vi "Create Execution Unit.vi"(8 "error in":errorcluster, 10 "Item Ref":T2=18446744073709551615 format="%.0x", 11 "Execution Unit Factory Implementation in":refnum<class "Execution Unit Factory.lvclass">) -> (0 "error out":errorcluster, 1 "Asynchronous Execution Units":cluster{"Grouped Execution Units":T1[]}[](array[cluster]) {"Grouped Execution Units"."ReadWrite Channels" format="%.0x"; "Grouped Execution Units"."Outgoing Channels" format="%.0x"; "Grouped Execution Units"."Incoming Channels" format="%.0x"}, 2 "Inline Execution Units":T1[](array[typedef]) {"ReadWrite Channels" format="%.0x"; "Outgoing Channels" format="%.0x"; "Incoming Channels" format="%.0x"}, 3 "Execution Unit Factory Implementation out":refnum<class "Execution Unit Factory.lvclass">)   [LabVIEW 2020, in "Ballard ARINC 429 Engine.lvlib" / "Implementation.lvlib" / "Execution Unit Factory.lvclass"]
uses:
  Execution Unit Factory.lvclass
  Interfaces/Execution Unit/Execution Unit.lvclass
  <vilib>/NI VeriStand/Custom Device API/Custom Device Item Ref.ctl
  <vilib>/NI VeriStand/Custom Device API/Custom Device API.lvlib
  Interfaces/Controls/Execution Unit Information.ctl
  Interfaces/Interfaces.lvlib
  Rx Execution Unit/Rx Execution Unit.lvclass
  System Explorer/Implementation/Implementation.lvlib
  Tx Acyclic Labels Execution Unit/Tx Acyclic Labels Execution Unit.lvclass
  Scripting/Ballard/Ballard ARINC 429 Scripting.lvlib
  Custom Device/Custom Device.lvlib
  Tx Scheduled Labels Execution Unit/Tx Scheduled Labels Execution Unit.lvclass
  C:/Users/nitest/Desktop/Git 2020/niveristand-ballard-arinc429-custom-device/Source/Custom Device Support/Engine/Implementation/Execution Unit/Execution Unit.lvclass
  C:/Users/nitest/Desktop/Git 2020/niveristand-ballard-arinc429-custom-device/Source/Custom Device Support/Engine/Interfaces/Execution Unit/Execution Unit.lvclass
  C:/Users/nitest/Desktop/Git 2020/niveristand-ballard-arinc429-custom-device/Source/Custom Device Support/Engine/Implementation/Rx Execution Unit/Rx Execution Unit.lvclass
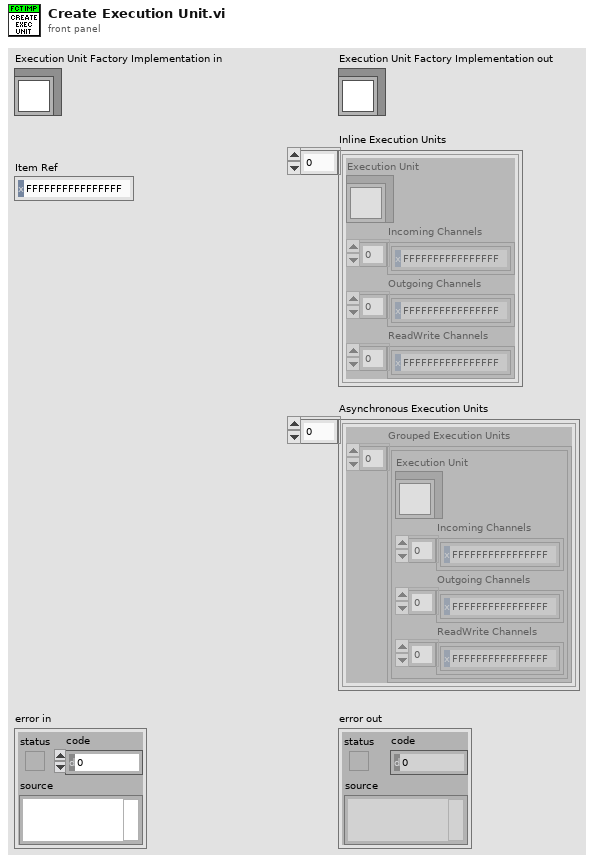
[diagram p1: front panel]
types:
  T1 = typedef "Ballard ARINC 429 Engine.lvlib/Interfaces.lvlib/Execution Unit Information.ctl" = cluster{"Execution Unit":refnum<class "Execution Unit.lvclass">, "Incoming Channels":T2[], "Outgoing Channels":T2[], "ReadWrite Channels":T2[]}
  T2 = typedef "Custom Device API.lvlib/Custom Device Item Ref.ctl" = u64
  T3 = typedef "RT Hardware Channel Settings.ctl" = cluster{"channel #":u16, "channel handle":u64, "labels settings for RT":T4[]}
  T4 = typedef "RT Label Settings.ctl" = cluster{"Name":string, "xmlName":string, "label":T5, "transfer period":u32, "SDI_Enabled":bool, "SDI":u8, "parameter driver data":T6, "transfer type":T9, "has timestamp?":bool, "Label Disable/Trigger Channel Reference":T2, "Message Handle":u64, "Initialized?":bool, "Word Initial Raw Value":u32, "Label Timestamp Channel Data Reference":T10, "disabled":bool}
  T5 = typedef "Label.ctl" = u8
  T6 = typedef "RT Parameters.ctl" = cluster{"parameter definitions":T7[], "Tx parameter refs":T2[]}
  T7 = typedef "Parameter Definition.ctl" = cluster{"start index":i32, "size":i32, "encoding":T8, "signed":bool, "scale multiplier":dbl, "scale offset":dbl}
  T8 = typedef "Encoding and Decoding.lvlib/Encoding.ctl" = enum16{"BNR", "BCD", "Discrete"}
  T9 = typedef "Transfer Type.ctl" = enum16{"Scheduled", "Acyclic", "Block", "Strobe"}
  T10 = typedef "Custom Device API.lvlib/Data Reference.ctl" = i32
  T11 = typedef "Rx Channel Data Offsets.ctl" = cluster{"error counts":u32, "rx execution time":i64}
  T12 = typedef "Custom Device API.lvlib/Custom Device Item Info.ctl" = cluster{"Name":string, "Is Channel":bool, "GUID":string, "Is Waveform":bool}
  T13 = cluster{"transfer type":T9, "Name":string, "hardware channel data":T3[], "Outgoing Channels":T2[], "ReadWrite Channels":T2[]}[]
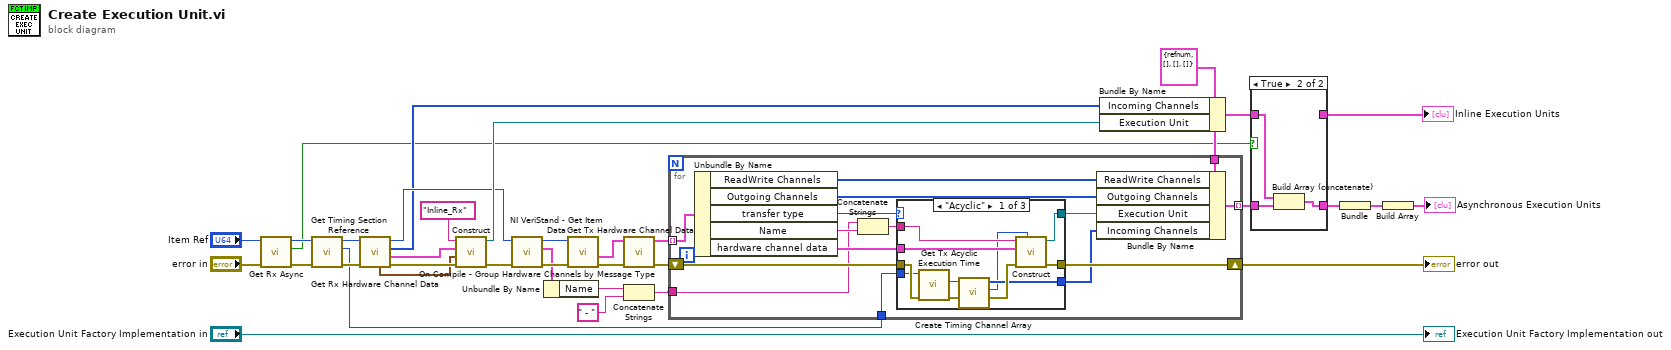
[diagram p0: block diagram]
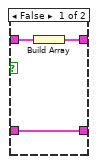
[diagram p2: hidden frame]
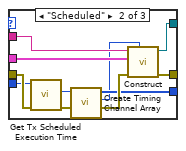
[diagram p3: hidden frame]
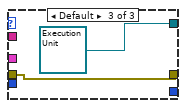
[diagram p4: hidden frame]
diagram:
  w23 = T1 {"Execution Unit"=refnum, "Incoming Channels"=[], "Outgoing Channels"=[], "ReadWrite Channels"=[]} ("Execution Unit Information")
  n1 = call "Get Rx Async.vi"("error in"="error in", "Ballard ARINC 429 custom device in"="Item Ref") -> ("error out"=w7:errorcluster, "rx async?"=w5:bool, "Ballard ARINC 429 custom device out"=w8:T2)  [unwired: 7 in]
  n2 = call "Get Timing Section Reference.vi"("error in"=w7, "Ballard ARINC 429 ref"=w8) -> ("error out"=w12:errorcluster, "timing section ref"=w9:T2, "Ballard ARINC 429 ref out"=w11:T2)  [unwired: 6 in, 1 out]
  n3 = call "Get Rx Hardware Channel Data.vi"("error in"=w12, "custom device ref in"=w11) -> ("error out"=w28:errorcluster, "Rx hardware channel data"=w29:T3[], "incoming channels"=w14:T2[], "custom device ref out"=w21:T2, "channel data offsets"=w13:T11)  [unwired: 5 in]
  n4 = call "Construct.vi"("error in"=w28, "channel data offsets"=w13, "RT hardware channels"=w29, "ID"="Inline_Rx") -> ("error out"=w22:errorcluster, "Ballard ARINC-429 Rx Execution Unit"=w27:refnum<class "Rx Execution Unit.lvclass">)  [unwired: 6 in]
  n5 = call <vilib>:"NI VeriStand - Get Item Data.vi"("error in (no error)"=w22, "Item Ref in"=w21) -> ("error out"=w19:errorcluster, "Item Info"=w18:T12, "Item Ref out"=w20:T2)  [unwired: 6 in, 1 out]
  n6 = Unbundle By Name(w18) -> ("Name"=w17:string)
  n7 = call "Get Tx Hardware Channel Data.vi"("error in"=w19, "custom device ref in"=w20) -> ("error out"=w31:errorcluster, "Tx hardware channel data"=w30:T3[])  [unwired: 6 in, 2 out]
  n8 = call "On Compile - Group Hardware Channels by Message Type.vi"("error in"=w31, "hardware channel data"=w30) -> ("error out"=w26:errorcluster, "hardware channel data by transfer type"=w24:T13)  [unwired: 8 in]
  n9 = Concatenate Strings(w17, " - " ("string")) -> (w15:string)
  n10 = for {
    shift-right: [w49] -> w25
    shift-left: w26 -> [w50]
    tunnel: w24 -> [w48] mode=indexing
    tunnel: w23 -> [w46]
    tunnel: [w44] -> w2 mode=indexing
    tunnel: w15 -> [w39]
    tunnel: w9 -> [w37]
    n11 = Unbundle By Name(w48) -> ("ReadWrite Channels"=w43:T2[], "Outgoing Channels"=w42:T2[], "transfer type"=w45:T9, "Name"=w40:string, "hardware channel data"=w41:T3[])
    n12 = Concatenate Strings(w39, w40) -> (w38:string)
    n13 = case shown="\"Acyclic\"" w45 {
      tunnel: w41 -> [w60 w70 _]
      tunnel: [w59 w69 refnum<class "Execution Unit.lvclass"> refnum ("Execution Unit")] -> w47
      tunnel: w50 -> [w56 w66 w71]
      tunnel: [w58 w68 w71] -> w49
      tunnel: w38 -> [w57 w67 _]
      tunnel: w37 -> [w55 w65 _]
      tunnel: [w52 w62 _] -> w36
      frame "Acyclic" {
        n14 = call "Get Tx Acyclic Execution Time.vi"("error in"=w56, "timing section in"=w55) -> ("error out"=w54:errorcluster, "tx acyclic execution time ref"=w53:T2)  [unwired: 7 in, 1 out]
        n15 = call "Create Timing Channel Array.vi"("timing channel ref"=w53) -> ("channel offset"=w51:i64, "timing channel ref array"=w52:T2[])  [unwired: 9 in]
        n16 = call "Construct.vi"("timing channel offset"=w51, "error in"=w54, "RT hardware channels"=w60, "ID"=w57) -> ("error out"=w58:errorcluster, "Ballard ARINC-429 Tx Acyclic execution unit out"=w59:refnum<class "Tx Acyclic Labels Execution Unit.lvclass">)  [unwired: 6 in]
      }
      frame "Scheduled" {
        n17 = call "Get Tx Scheduled Execution Time.vi"("error in"=w66, "timing section in"=w65) -> ("error out"=w64:errorcluster, "tx scheduled execution time ref"=w63:T2)  [unwired: 7 in, 1 out]
        n18 = call "Create Timing Channel Array.vi"("timing channel ref"=w63) -> ("channel offset"=w61:i64, "timing channel ref array"=w62:T2[])  [unwired: 9 in]
        n19 = call "Construct.vi"("timing channel offset"=w61, "error in"=w64, "RT hardware channels"=w70, "ID"=w67) -> ("error out"=w68:errorcluster, "Ballard ARINC-429 Tx Execution Unit out"=w69:refnum<class "Tx Scheduled Labels Execution Unit.lvclass">)  [unwired: 6 in]
      }
      frame Default {
      }
    }
    n20 = Bundle By Name(cluster=w46, "ReadWrite Channels"=w43, "Outgoing Channels"=w42, "Execution Unit"=w47, "Incoming Channels"=w36) -> (w44:T1)
  }
  "error out" <- w25
  n21 = Bundle By Name(cluster=w23, "Incoming Channels"=w14, "Execution Unit"=w27) -> (w34:T1)
  n22 = case shown="True" w5 {
    tunnel: w34 -> [w75 w77]
    tunnel: [w74 _] -> w33
    tunnel: w2 -> [w73 w78]
    tunnel: [w73 w76] -> w1
    frame False {
      n23 = Build Array(w75) -> (w74:T1[])
    }
    frame True {
      n24 = Build Array (concatenate)(w77, w78) -> (w76:T1[])
    }
  }
  "Inline Execution Units" <- w33
  n25 = Bundle(w1) -> (w4:cluster{T1[]})  [unwired: 1 in]
  n26 = Build Array(w4) -> (→"Asynchronous Execution Units":cluster{T1[]}[])
  "Execution Unit Factory Implementation out" <- "Execution Unit Factory Implementation in"
